vi "Variable glob mails.vi"() -> ()   [LabVIEW 2022 SP3]
panel:
  out "Domaine mail labo":string
  out "Noms station":string[](array[string])
  out "Retour":string
  out "Serveur":string
  in  "Mails envoi":string[](array[string])
  in  "Mails dispo":string[](array[string])
  in  "Mails IAS noms":string[](array[string])
  in  "Mails autres":string[](array[string])
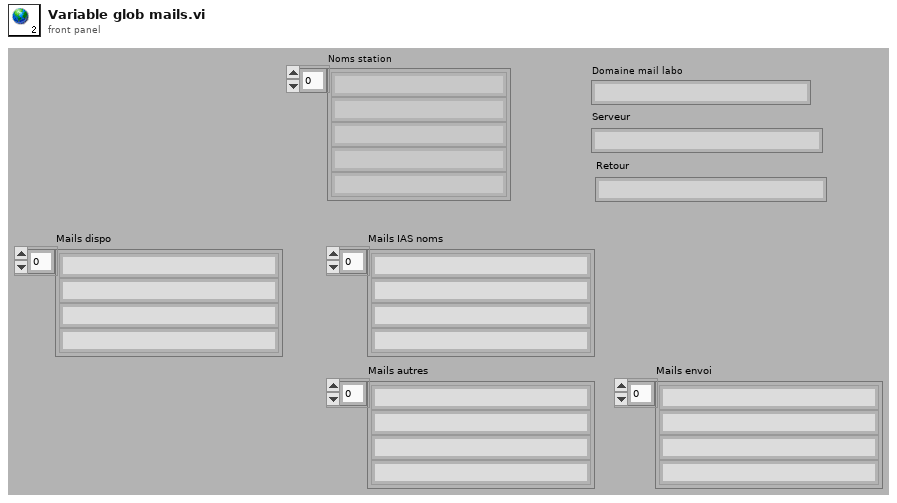
[diagram p1: front panel]
diagram:
